vi "Set All NI-SWITCH Properties.vi"(8 "error in":errorcluster, 10 "properties":T1, 11 "ni-switch custom device in":T2 format="%.0x") -> (0 "error out":errorcluster, 3 "ni-switch custom device out":T2 format="%.0x")   [LabVIEW 2020, in "NI-SWITCH Scripting.lvlib"]
uses:
  NI-SWITCH Scripting.lvlib
  <vilib>/NI VeriStand/Custom Device API/Custom Device Item Ref.ctl
  NI-SWITCH All Properties.ctl
  <vilib>/NI VeriStand/Custom Device API/Custom Device API.lvlib
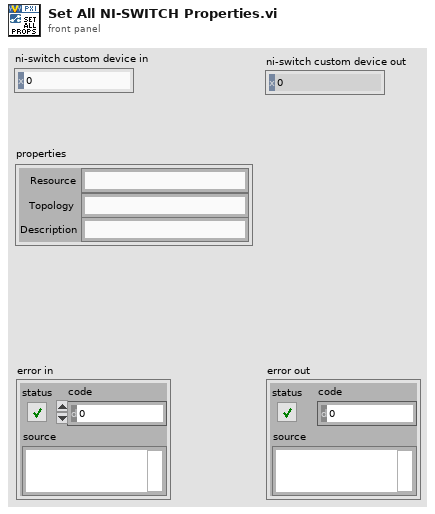
[diagram p1: front panel]
types:
  T1 = typedef "NI-SWITCH Scripting.lvlib/NI-SWITCH All Properties.ctl" = cluster{"Resource":string, "Topology":string, "Description":string}
  T2 = typedef "Custom Device API.lvlib/Custom Device Item Ref.ctl" = u64
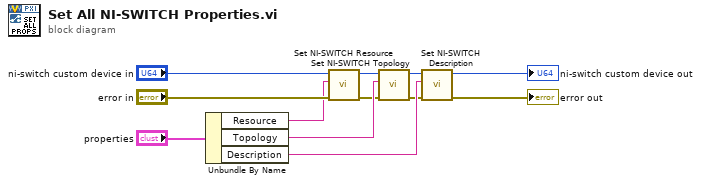
[diagram p0: block diagram]
diagram:
  n1 = Unbundle By Name("properties") -> ("Resource"=w9:string, "Topology"=w6:string, "Description"=w8:string)
  n2 = call "Set NI-SWITCH Resource.vi"("error in"="error in", "resource"=w9, "ni-switch custom device in"="ni-switch custom device in") -> ("error out"=w2:errorcluster, "ni-switch custom device out"=w1:T2)  [unwired: 7 in]
  n3 = call "Set NI-SWITCH Topology.vi"("error in"=w2, "topology"=w6, "ni-switch custom device in"=w1) -> ("error out"=w7:errorcluster, "ni-switch custom device out"=w5:T2)  [unwired: 7 in]
  n4 = call "Set NI-SWITCH Description.vi"("error in"=w7, "description"=w8, "ni-switch custom device in"=w5) -> ("error out"=→"error out":errorcluster, "ni-switch custom device out"=→"ni-switch custom device out":T2)  [unwired: 7 in]
